vi "Convert Activation Event.vi"(8 "error in":errorcluster, 11 "Activation Event Args":T3) -> (0 "error out":errorcluster, 3 "Activation":T1)   [LabVIEW 2026, in "ToastNotification.lvlib" / "ToastService.lvclass"]
doc: "Convert borrowed toolkit activation event arguments into LabVIEW strings and key/value pairs. Read Argument, acquire UserInput, enumerate its entries and close that acquired collection on every path. Never close Activation Event Args. Stop conversion on the first error; return that error separately from Activation. Partial data may be returned on failure."
uses:
  ToastService.lvclass
  Reflection DotNet/Callback Object Reference.ctl
  ToastNotification/Activation.ctl
  ToastNotification/Argument.ctl
  Reflection DotNet/Reflection DotNet.lvlib
  ToastNotification/ToastNotification.lvlib
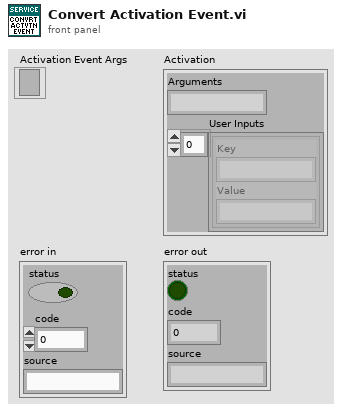
[diagram p1: front panel]
types:
  T1 = typedef "ToastNotification.lvlib/Activation.ctl" = cluster{"Arguments":string, "User Inputs":T2[]}
  T2 = typedef "ToastNotification.lvlib/Argument.ctl" = cluster{"Key":string, "Value":string}
  T3 = typedef "ToastNotification.lvlib/Reflection DotNet.lvlib/Callback Object Reference.ctl" = refnum<k24>
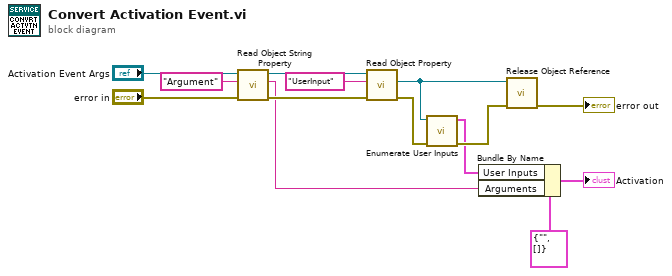
[diagram p0: block diagram]
diagram:
  n1 = call "Read Object String Property.vi"("error in"="error in", "property name"="Argument", "object in"="Activation Event Args") -> ("error out"=w8:errorcluster, "text"=w2:string, "object out"=w4:T3)  [unwired: 6 in]
  n2 = call "Read Object Property.vi"("error in"=w8, "property name"="UserInput", "object in"=w4) -> ("error out"=w7:errorcluster, "value"=w6:T3)  [unwired: 6 in, 1 out]
  n3 = call "Enumerate User Inputs.vi"("error in"=w7, "User Input Collection"=w6) -> ("error out"=w10:errorcluster, "Entries"=w1:cluster{"Key":string, "Value":string}[])  [unwired: 8 in]
  n4 = Bundle By Name(cluster=T1 {"Arguments"="", "User Inputs"=[]}, "User Inputs"=w1, "Arguments"=w2) -> (→"Activation":T1)
  n5 = call "Release Object Reference.vi"("error in"=w10, "object"=w6) -> ("error out"=→"error out":errorcluster)  [unwired: 9 in]
